vi "Connection Local IP.vi"(8 "error in (no error)":errorcluster, 11 "Processing in":refnum<class "Processing.lvclass">) -> (0 "error out":errorcluster, 2 "local IP":string, 3 "Processing out":refnum<class "Processing.lvclass">)   [LabVIEW 2020, in "MCP Server.lvlib" / "MCP Connection Probe.lvclass"]
doc: "Returns the local IP address of the TCP connection a request arrived on, as a dotted IPv4 string (for example 127.0.0.1). This is the address of this computer that the client connected to, not the client's address.\n\nWhy: Check Client Access.vi decides \"this computer only\" from it instead of from the client's reverse-DNS name, which can be spoofed. A local address of 127.x means the connection arrived over loopback. On Windows' strong host model a remote peer cannot produce a connection whose local address is a loopback address. A client on this computer that connects through the LAN IP gets the LAN IP, not 127.x.\n\nHow: the connection is taken from Processing in (HTTP Server Processing:Get Connection), cast to Stream-TCP TCP Client and read through its protected Get TCP Connection, which is why this VI is a member of MCP Connection Probe.lvclass, a child of TCP Client. The address comes from TCP Get Local IP.vi (NI_FTP). No DNS lookup is made.\n\nOn error (a connection that is not a TCP client, an invalid refnum, or an error at error in) local IP is empty and the error goes to error out."
uses:
  MCP Connection Probe.lvclass
  <vilib>/IlluminatedG/IG HTTP Server/HTTP Server/Processing/Processing.lvclass
  <vilib>/IlluminatedG/lv-stream-tcp/TCP Client/TCP Client.lvclass
  <vilib>/IlluminatedG/IG HTTP Server/HTTP Server/Processing/Processing.lvclass/Processing.ctl
  <vilib>/FTP/NI_FTP.lvlib
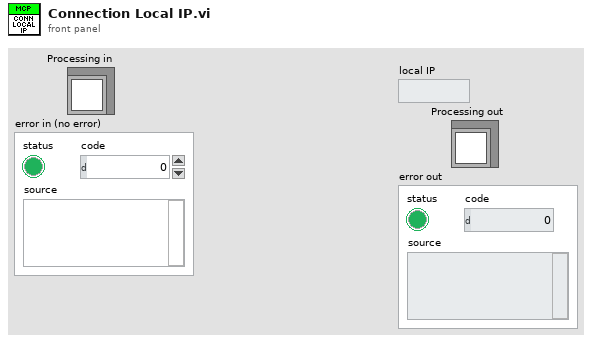
[diagram p1: front panel]
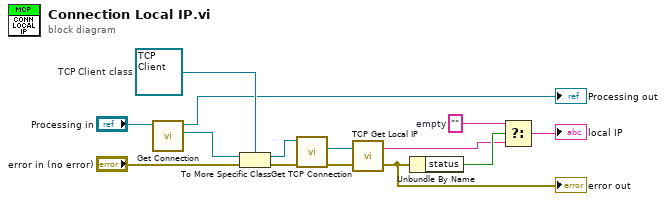
[diagram p0: block diagram]
diagram:
  w5 = ""  # empty
  w12 = refnum<class "TCP Client.lvclass"> refnum  # TCP Client class
  n1 = call <vilib>:"Get Connection.vi"("Processing in"="Processing in") -> ("Connection"=w13:refnum<class "HTTP TCP Client.lvclass">, "Processing out"=→"Processing out":refnum<class "Processing.lvclass">)  [unwired: 9 in]
  n2 = To More Specific Class(target class=w12, reference=w13, error in="error in (no error)") -> (specific class reference=w10:refnum<class "TCP Client.lvclass">, error out=w9:errorcluster)
  n3 = call <vilib>:"Get TCP Connection.vi"("error in (no error)"=w9, "TCP Client in"=w10) -> ("error out"=w7:errorcluster, "TCP Connection"=w8:refnum<k5>)  [unwired: 7 in, 1 out]
  n4 = call <vilib>:"TCP Get Local IP.vi"("error in (no error)"=w7, "connectionID"=w8) -> ("error out"=w1:errorcluster, "IP"=w4:string)
  "error out" <- w1
  n5 = Unbundle By Name(w1) -> ("status"=w6:bool)
  n6 = Select(t=w5, s=w6, f=w4) -> (s? t:f=→"local IP":string)
